vi "Test_RouteGuide_BidirectionalStreaming.vi"() -> (0 "Array of Error Description":T1)   [LabVIEW 2019]
uses:
  gRPC_ATS/TestUtility/utility.llb/array of error description.ctl
  gRPC_ATS/TestUtility/utility.llb/error description.ctl
  gRPC_ATS/TestUtility/utility.llb/error type.ctl
  examples/route_guide/route_guide_client/RPC Messages/routeguide_RouteNote.ctl
  examples/route_guide/route_guide_client/RPC Messages/routeguide_Point.ctl
  examples/route_guide/route_guide_client/route_guide_client.lvlib
panel:
  out "Pass":bool
  in  "Client VI Path":path=path "../../examples/route_guide/route_guide_client/Bidirectional Streaming RouteGuide Test.vi"
  in  "Server VI path":path=path "../../examples/route_guide/route_guide_server/Run Service.vi"
  in  "error in":errorcluster
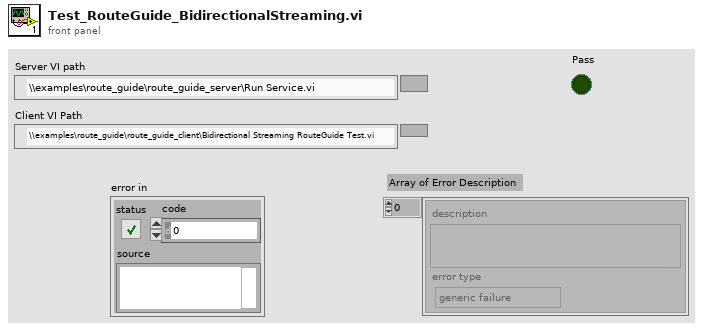
[diagram p1: front panel]
types:
  T1 = typedef "array of error description.ctl" = T2[]
  T2 = typedef "error description.ctl" = cluster{"description":string, "error type":T3}
  T3 = typedef "error type.ctl" = enum32{"generic failure", "boundary case", "precision", "expected error"}
  T4 = typedef "route_guide_client.lvlib/routeguide_RouteNote.ctl" = cluster{"location":T5, "message":string}
  T5 = typedef "route_guide_client.lvlib/routeguide_Point.ctl" = cluster{"latitude":i32, "longitude":i32}
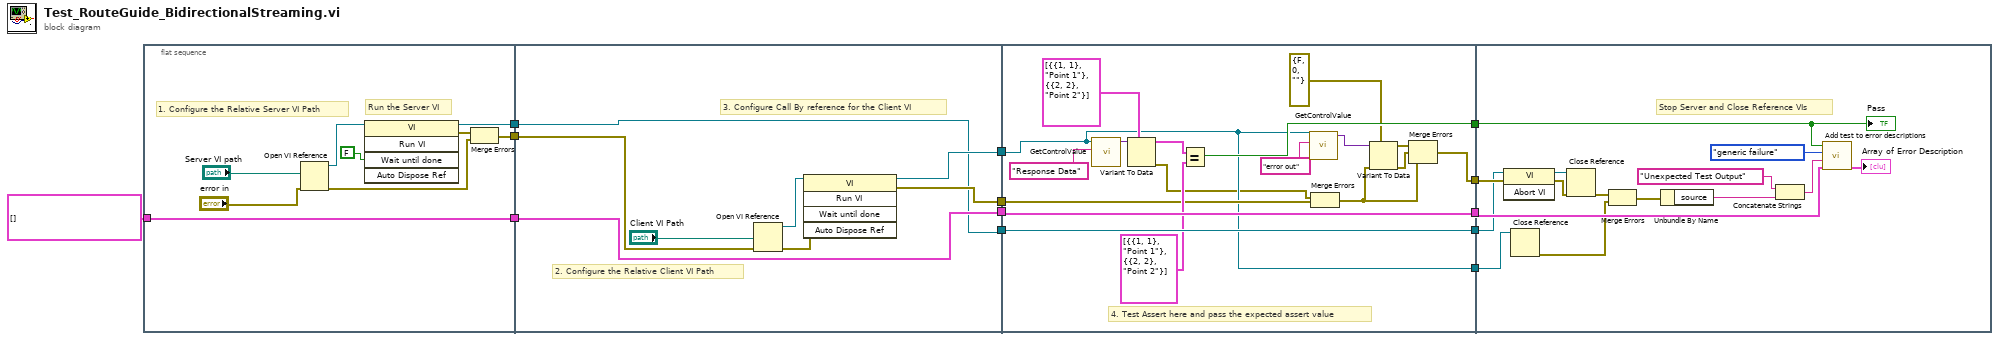
[diagram p0: block diagram]
diagram:
  n1 = flat-sequence {
    tunnel: T1 [] ("error descriptions in") -> [w18]
    tunnel: [w18] -> w13
    tunnel: [w17] -> w12
    tunnel: [w14] -> w11
    tunnel: w13 -> [w29]
    tunnel: [w29] -> w10
    tunnel: w12 -> [w23]
    tunnel: w11 -> [w28]
    tunnel: [w23] -> w5
    tunnel: [w25] -> w3
    tunnel: [w24] -> w2
    tunnel: w10 -> [w48]
    tunnel: [w48] -> w9
    tunnel: [w33] -> w8
    tunnel: [w46] -> w6
    tunnel: w5 -> [w47]
    tunnel: [w47] -> w4
    tunnel: w3 -> [w40]
    tunnel: w2 -> [w36]
    tunnel: [w36] -> w1
    tunnel: w9 -> [w58]
    tunnel: w8 -> [w55]
    tunnel: w6 -> [w54]
    tunnel: w4 -> [w50]
    tunnel: w1 -> [w49]
    frame #0 {
      # "1. Configure the Relative Server VI Path"
      # "Run the Server VI"
      n2 = Open VI Reference(vi path="Server VI path", error in (no error)="error in") -> (vi reference=w20:refnum<vi>, error out=w16:errorcluster)  [unwired: 4 in]
      n3 = invoke class="VI" method="Run VI"(reference=w20, "Wait until done"=FALSE ("Wait Until Done")) -> (reference out=w17:refnum<vi>, error out=w15:errorcluster)  [unwired: 3 in, 3 out]
      n4 = Merge Errors(w15, w16) -> (w14:errorcluster)
    }
    frame #1 {
      # "2. Configure the Relative Client VI Path"
      # "3. Configure Call By reference for the Client VI"
      n5 = Open VI Reference(vi path="Client VI Path", error in (no error)=w28) -> (vi reference=w26:refnum<vi>, error out=w27:errorcluster)  [unwired: 4 in]
      n6 = invoke class="VI" method="Run VI"(reference=w26, error in=w27) -> (reference out=w24:refnum<vi>, error out=w25:errorcluster)  [unwired: 3 in, 3 out]
    }
    frame #2 {
      # "4. Test Assert here and pass the expected assert value"
      n7 = call "GetControlValue.vi"("Control Label"="Response Data", "VI Reference"=w36) -> ("Value"=w44:variant)  [unwired: 8 in, 1 out]
      n8 = Variant To Data(type=T4[] [{"location"={"latitude"=1, "longitude"=1}, "message"="Point 1"}, {"location"={"latitude"=2, "longitude"=2}, "message"="Point 2"}] ("Response Data"), Variant=w44) -> (data=w42:T4[], error out=w32:errorcluster)  [unwired: 1 in]
      n9 = Equal?(x=w42, y=T4[] [{"location"={"latitude"=1, "longitude"=1}, "message"="Point 1"}, {"location"={"latitude"=2, "longitude"=2}, "message"="Point 2"}] ("Response Data")) -> (x = y?=w46:bool)
      n10 = call "GetControlValue.vi"("Control Label"="error out", "VI Reference"=w36) -> ("Value"=w38:variant)  [unwired: 8 in, 1 out]
      n11 = Merge Errors(w32, w40) -> (w34:errorcluster)
      n12 = Variant To Data(error in=w34, type=errorcluster {"status"=FALSE, "code"=0, "source"=""} ("error constant"), Variant=w38) -> (data=w31:errorcluster, error out=w35:errorcluster)
      n13 = Merge Errors(w31, w35, w34) -> (w33:errorcluster)
    }
    frame #3 {
      # "Stop Server and Close Reference VIs"
      n14 = invoke class="VI" method="Abort VI"(reference=w50, error in=w55) -> (reference out=w56:refnum<vi>, error out=w57:errorcluster)  [unwired: 1 in, 1 out]
      n15 = Close Reference(reference=w49) -> (error out=w52:errorcluster)  [unwired: 1 in]
      n16 = Close Reference(reference=w56, error in (no error)=w57) -> (error out=w53:errorcluster)
      n17 = Merge Errors(w53, w52) -> (w51:errorcluster)
      n18 = Unbundle By Name(w51) -> ("source"=w60:string)
      n19 = Concatenate Strings("Unexpected Test Output" ("string"), w60) -> (w61:string)
      n20 = call "Add test to error descriptions.vi"("error descriptions in"=w58, "error string"=w61, "error type"=error_type."generic failure", "pass"=w54) -> ("error description out"=→"Array of Error Description":T1)  [unwired: 3 in]
      "Pass" <- w54
    }
  }
